vi "Test Mutex.vi"() -> ()   [LabVIEW 2013]
uses:
  <vilib>/LabVIEW Open Source Project/MQTT Control Packets/Control Packets/ControlPacket/Control Packet Type -- enum.ctl
  <vilib>/LabVIEW Open Source Project/MQTT Control Packets/Control Packets/CONNACK/Connect Return Code -- enum.ctl
  <vilib>/LabVIEW Open Source Project/MQTT Control Packets/Control Packets/ControlPacket/ControlPacket.lvclass
  <vilib>/LabVIEW Open Source Project/MQTT Control Packets/Control Packets/PUBLISH/PUBLISH.lvclass
  source/Client class/Client.lvclass
  <vilib>/LabVIEW Open Source Project/MQTT Connection/MQTT_Base/Base Class/MQTT_Base.lvclass
  <vilib>/LabVIEW Open Source Project/MQTT Control Packets/Control Packets/CONNACK/CONNACK.lvclass
  <vilib>/LabVIEW Open Source Project/Connection/Connection.TCP/Connection.TCP.lvclass
  <vilib>/LabVIEW Open Source Project/Connection/Connection/Connection.lvclass
panel:
  out "Return Code 2":T1=enum."Server Unavailable"
  out "Return Code":T1=enum."Server Unavailable"
  out "Array 2":string[](array[string])
  out "Array":T2[](array[typedef])
  out "server connected":bool
  out "listener error":errorcluster
  out "server session error":errorcluster
  out "error out":errorcluster
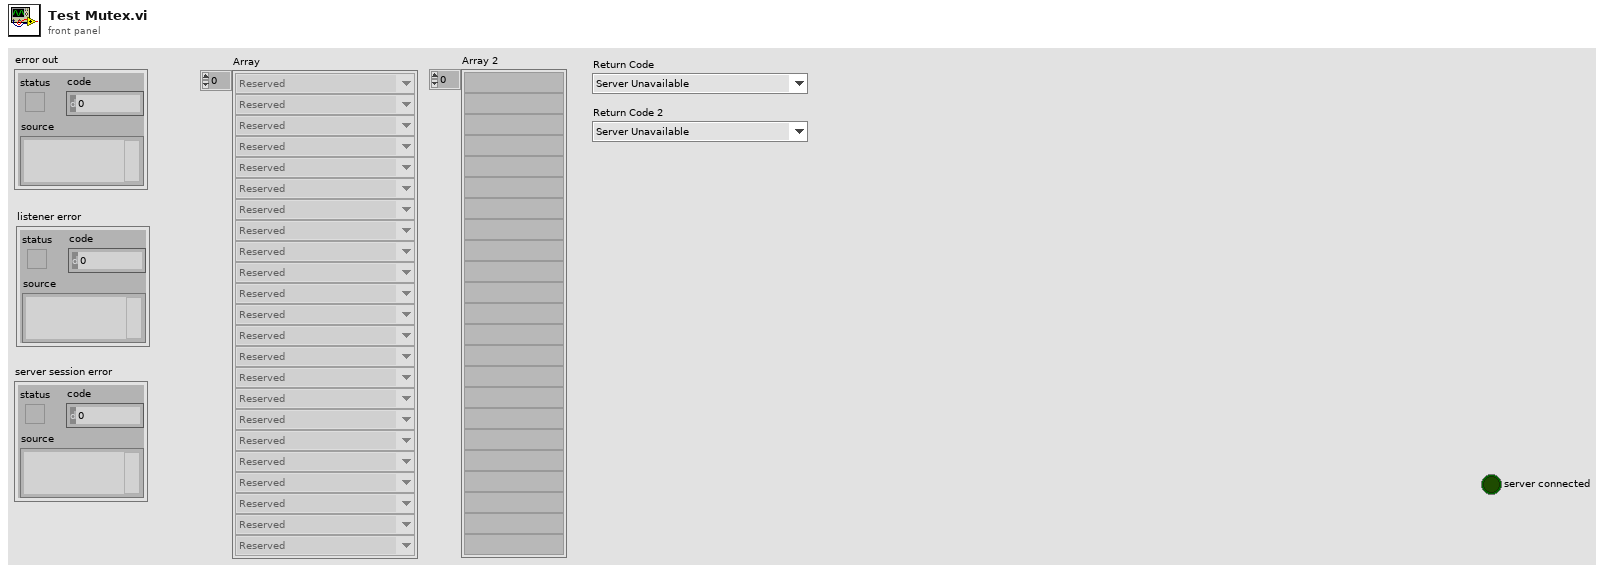
[diagram p1: front panel]
types:
  T1 = typedef "MQTT_Control_Packets.lvlib/CONNACK.lvclass/Connect Return Code -- enum.ctl" = enum16{"Connection accepted", "Unacceptable protocol version", "Identifier Rejected", "Server Unavailable", "Bad Username or Password", "Not Authorized"}
  T2 = typedef "MQTT_Control_Packets.lvlib/ControlPacket.lvclass/Control Packet Type -- enum.ctl" = enum16{"Reserved", "CONNECT", "CONNACK", "PUBLISH", "PUBACK", "PUBREC", "PUBREL", "PUBCOMP", "SUBSCRIBE", "SUBACK", "UNSUBSCRIBE", "UNSUBACK", "PINGREQ", "PINGRESP", "DISCONNECT", "AUTH"}
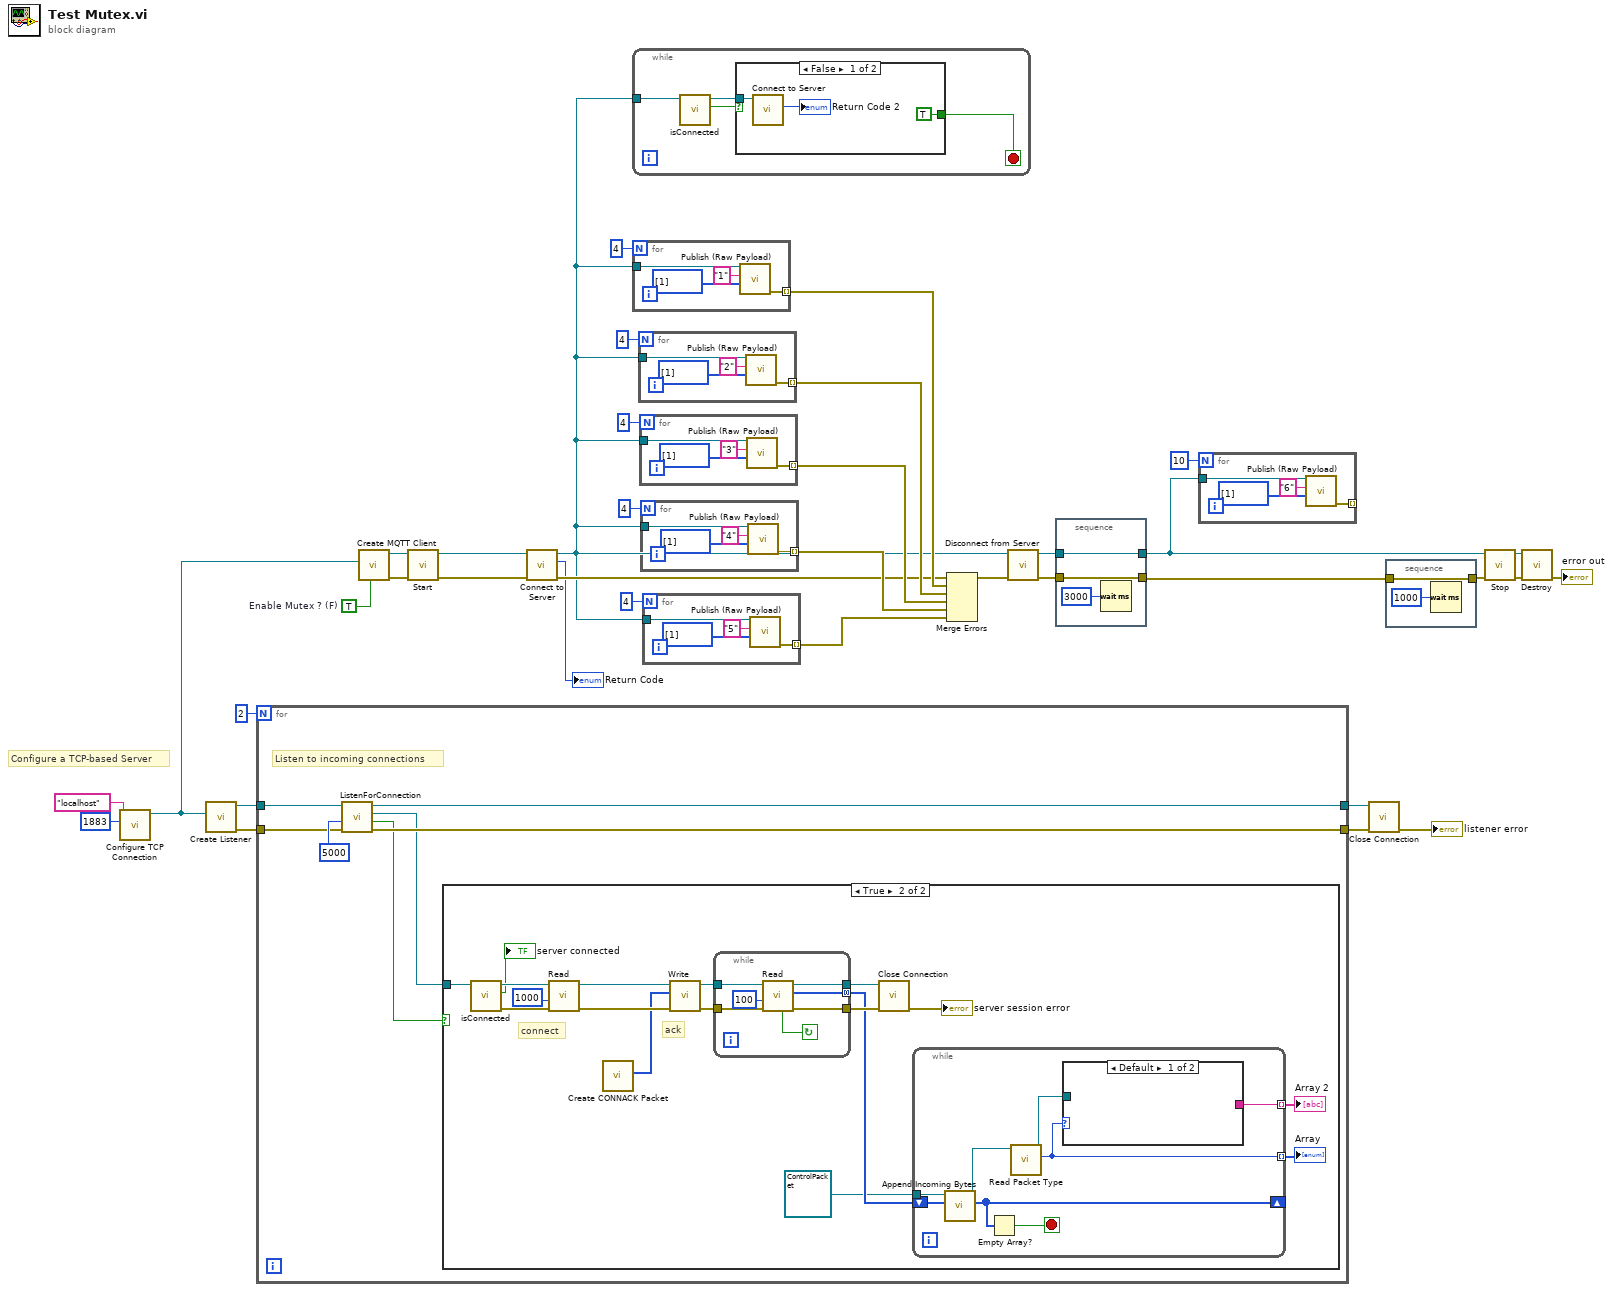
[diagram p0: block diagram]
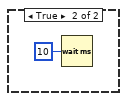
[diagram p2: hidden frame]
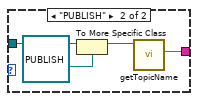
[diagram p4: hidden frame]
diagram:
  w21 = TRUE  # Enable Mutex ? (F)
  # "Configure a TCP-based Server"
  n1 = call <vilib>:"Configure TCP Connection.vi"("remote port (80)"=u16 1883, "address (localhost)"="localhost") -> ("Connection.TCP"=w23:refnum<class "Connection.TCP.lvclass">)  [unwired: 8 in, 1 out]
  n2 = call <vilib>:"Create Listener.vi"("Connection Configuration"=w23) -> ("error out"=w28:errorcluster, "Listener"=w30:refnum<class "Connection.TCP.lvclass">)  [unwired: 9 in]
  n3 = for {
    N: 2 -> [_]
    tunnel: w30 -> [w44]
    tunnel: [w42] -> w29
    tunnel: w28 -> [w41]
    tunnel: [w40] -> w27
    # "Listen to incoming connections"
    n4 = call <vilib>:"ListenForConnection.vi"("error in (no error)"=w41, "timeout (2000 ms)"=5000 ("bytes to read (100)"), "Listener"=w44) -> ("error out"=w40:errorcluster, "New connection"=w38:bool, "Connection"=w39:refnum<class "Connection.lvclass">, "Listener out"=w42:refnum<class "Connection.TCP.lvclass">)  [unwired: 5 in]
    n5 = case shown="True" w38 {
      tunnel: w39 -> [_ w57]
      frame False {
      }
      frame True {
        # "ack"
        # "connect"
        n6 = call <vilib>:"isConnected.vi"("Connection in"=w57) -> ("error out"=w55:errorcluster, "connected"=→"server connected":bool, "Connection out"=w56:refnum<class "Connection.lvclass">)  [unwired: 8 in]
        n7 = call <vilib>:"Read.vi"("error in (no error)"=w55, "timeout (2000 ms)"=1000 ("bytes to read (100)"), "TCPConnection in"=w56) -> ("error out"=w59:errorcluster, "TCPConnection out"=w60:refnum<class "Connection.lvclass">)  [unwired: 4 in, 3 out]
        n8 = call <vilib>:"Create CONNACK Packet.vi"() -> ("Bytes Stream"=w53:u8[])  [unwired: 9 in, 2 out]
        n9 = call <vilib>:"Write.vi"("error in (no error)"=w59, "Bytes"=w53, "Connection in"=w60) -> ("error out"=w51:errorcluster, "Connection"=w52:refnum<class "Connection.lvclass">)  [unwired: 7 in]
        n10 = while {
          tunnel: w52 -> [w79]
          tunnel: w51 -> [w78]
          tunnel: [w77] -> w50
          tunnel: [w76] -> w49
          tunnel: [w75] -> w48 mode=concatenating
          stop <- w74 continue-if-true
          n11 = call <vilib>:"Read.vi"("error in (no error)"=w78, "timeout (2000 ms)"=100 ("bytes to read (100)"), "TCPConnection in"=w79) -> ("error out"=w76:errorcluster, "Bytes"=w75:u8[], "TCPConnection out"=w77:refnum<class "Connection.lvclass">, "connected"=w74:bool)  [unwired: 4 in, 1 out]
        }
        n12 = call <vilib>:"Close Connection.vi"("error in (no error)"=w49, "Connection in"=w50) -> ("error out"=→"server session error":errorcluster)  [unwired: 8 in, 1 out]
        n13 = while {
          tunnel: refnum<class "ControlPacket.lvclass"> refnum ("Incomplete ControlPacket") -> [w68]
          shift-right: [w67] -> _
          shift-left: w48 -> [w69]
          tunnel: [w64] -> w46 mode=indexing
          tunnel: [w62] -> w45 mode=indexing
          stop <- w66 stop-if-true
          n14 = call <vilib>:"Append Incoming Bytes.vi"("Incoming Packets"=w69, "Incomplete ControlPacket"=w68) -> ("Remaining Packets"=w67:u8[], "ControlPacket"=w65:refnum<class "ControlPacket.lvclass">)  [unwired: 6 in, 2 out]
          n15 = Empty Array?(array=w67) -> (empty?=w66:bool)
          n16 = call <vilib>:"Read Packet Type.vi"("ControlPacket in"=w65) -> ("Control Packet Type"=w64:T2, "ControlPacket out"=w63:refnum<class "ControlPacket.lvclass">)  [unwired: 9 in]
          n17 = case shown="Default" w64 {
            tunnel: w63 -> [_ w73]
            tunnel: [_ w70] -> w62
            frame Default {
            }
            frame "PUBLISH" {
              n18 = To More Specific Class(target class=refnum<class "PUBLISH.lvclass"> refnum ("PUBLISH in"), reference=w73) -> (specific class reference=w72:refnum<class "PUBLISH.lvclass">)  [unwired: 1 in, 1 out]
              n19 = call <vilib>:"getTopicName.vi"("PUBLISH in"=w72) -> ("Topic"=w70:string)  [unwired: 8 in, 2 out]
            }
          }
        }
        "Array" <- w46
        "Array 2" <- w45
      }
    }
  }
  n20 = call "Create MQTT Client.vi"("Enable Mutex ? (F)"=w21, "Connection Configuration"=w23) -> ("error out"=w36:errorcluster, "Client out"=w34:refnum<class "Client.lvclass">)  [unwired: 8 in]
  n21 = call <vilib>:"Start.vi"("error in (no error)"=w36, "MQTT_Base in"=w34) -> ("error out"=w35:errorcluster, "MQTT_Base out"=w33:refnum<class "Client.lvclass">)  [unwired: 7 in, 1 out]
  n22 = call "Connect to Server.vi"("error in (no error)"=w35, "Client in"=w33) -> ("error out"=w9:errorcluster, "Return Code"=→"Return Code":T1, "Client out"=w8:refnum<class "Client.lvclass">)  [unwired: 6 in, 1 out]
  n23 = while {
    tunnel: w8 -> [w84]
    stop <- w81 stop-if-true
    n24 = call <vilib>:"isConnected.vi"("Client in"=w84) -> ("connected"=w83:bool, "Client out"=w82:refnum<class "Client.lvclass">)  [unwired: 8 in, 1 out]
    n25 = case shown="False" w83 {
      tunnel: w82 -> [w87 _]
      tunnel: [TRUE _] -> w81
      frame False {
        n26 = call "Connect to Server.vi"("Client in"=w87) -> ("Return Code"=→"Return Code 2":T1)  [unwired: 7 in, 3 out]
      }
      frame True {
        n27 = Wait (ms)(milliseconds to wait=u32 10) -> ()  [unwired: 1 out]
      }
    }
  }
  n28 = for {
    N: 4 -> [_]
    tunnel: w8 -> [w90]
    tunnel: [w89] -> w10 mode=indexing
    n29 = call "Publish (Raw Payload).vi"("Binary Payload"=u8[] [1], "Topic Name"="1", "Client in"=w90) -> ("error out"=w89:errorcluster)  [unwired: 6 in, 2 out]
  }
  n30 = for {
    N: 4 -> [_]
    tunnel: w8 -> [w94]
    tunnel: [w93] -> w11 mode=indexing
    n31 = call "Publish (Raw Payload).vi"("Binary Payload"=u8[] [1], "Topic Name"="2", "Client in"=w94) -> ("error out"=w93:errorcluster)  [unwired: 6 in, 2 out]
  }
  n32 = for {
    N: 4 -> [_]
    tunnel: w8 -> [w98]
    tunnel: [w97] -> w12 mode=indexing
    n33 = call "Publish (Raw Payload).vi"("Binary Payload"=u8[] [1], "Topic Name"="3", "Client in"=w98) -> ("error out"=w97:errorcluster)  [unwired: 6 in, 2 out]
  }
  n34 = for {
    N: 4 -> [_]
    tunnel: w8 -> [w102]
    tunnel: [w101] -> w14 mode=indexing
    n35 = call "Publish (Raw Payload).vi"("Binary Payload"=u8[] [1], "Topic Name"="4", "Client in"=w102) -> ("error out"=w101:errorcluster)  [unwired: 6 in, 2 out]
  }
  n36 = for {
    N: 4 -> [_]
    tunnel: w8 -> [w106]
    tunnel: [w105] -> w13 mode=indexing
    n37 = call "Publish (Raw Payload).vi"("Binary Payload"=u8[] [1], "Topic Name"="5", "Client in"=w106) -> ("error out"=w105:errorcluster)  [unwired: 6 in, 2 out]
  }
  n38 = Merge Errors(w9, w10, w11, w12, w14, w13) -> (w20:errorcluster)
  n39 = call "Disconnect from Server.vi"("error in (no error)"=w20, "Client in"=w8) -> ("error out"=w22:errorcluster, "Client out"=w2:refnum<class "Client.lvclass">)  [unwired: 7 in, 1 out]
  n40 = stacked-sequence {
    tunnel: w22 -> [w110]
    tunnel: [w110] -> w4
    tunnel: [w109] -> w3
    tunnel: w2 -> [w109]
    frame #0 {
      n41 = Wait (ms)(milliseconds to wait=u32 3000) -> ()  [unwired: 1 out]
    }
  }
  n42 = for {
    N: 10 -> [_]
    tunnel: w3 -> [w113]
    tunnel: [w112] -> _ mode=indexing
    n43 = call "Publish (Raw Payload).vi"("Binary Payload"=u8[] [1], "Topic Name"="6", "Client in"=w113) -> ("error out"=w112:errorcluster)  [unwired: 6 in, 2 out]
  }
  n44 = call <vilib>:"Close Connection.vi"("error in (no error)"=w27, "Connection in"=w29) -> ("error out"=→"listener error":errorcluster)  [unwired: 8 in, 1 out]
  n45 = stacked-sequence {
    tunnel: w4 -> [w116]
    tunnel: [w116] -> w5
    frame #0 {
      n46 = Wait (ms)(milliseconds to wait=u32 1000) -> ()  [unwired: 1 out]
    }
  }
  n47 = call <vilib>:"Stop.vi"("error in (no error)"=w5, "MQTT_Base in"=w3) -> ("error out"=w31:errorcluster, "MQTT_Base out"=w32:refnum<class "Client.lvclass">)  [unwired: 7 in, 1 out]
  n48 = call <vilib>:"Destroy.vi"("error in (no error)"=w31, "MQTT_Base in"=w32) -> ("error out"=→"error out":errorcluster)  [unwired: 8 in, 1 out]
